vi "Confirm With User.vi"(8 "error in":errorcluster, 10 "message":string, 11 "key":string) -> (0 "error out":errorcluster, 1 "not supported?":bool, 2 "pending?":bool, 3 "confirmed?":bool)   [LabVIEW 2020, in "MCP Server.lvlib"]
doc: "Asks the user of the MCP client to confirm something (MCP elicitation without fields), for example before a tool deletes data or moves hardware. A wrapper around Ask User.vi with an empty requestedSchema.\n\nThe tool VI runs twice: on the first run pending? is TRUE - return at once and do NOTHING else, no side effects. On the second run confirmed? is TRUE when the user accepted; when it is FALSE (and pending? and not supported? are FALSE) the user declined or cancelled. not supported? is TRUE when the client cannot be asked (a legacy client, or no elicitation capability): fall back to a safe default or refuse.\n\nkey must be unique within the tool. See Ask User.vi for the details and the restrictions of form mode (never ask for passwords or keys)."
uses:
  MCP Server.lvlib
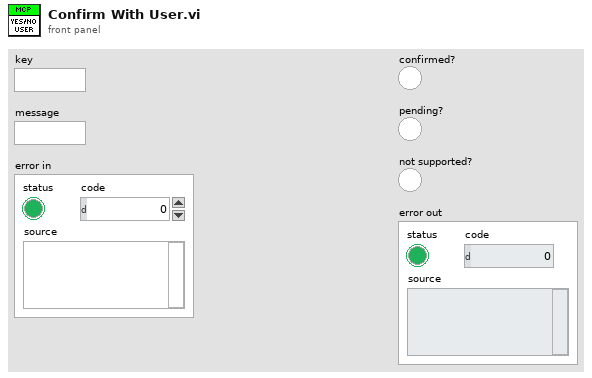
[diagram p1: front panel]
types:
  T1 = enum16{"accept", "decline", "cancel", "pending", "not supported"}
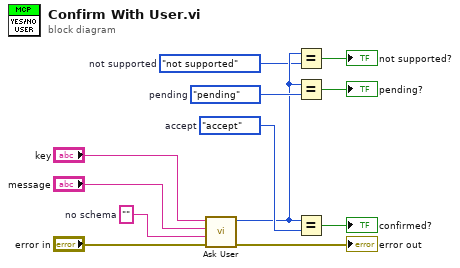
[diagram p0: block diagram]
diagram:
  w3 = T1."not supported"  # not supported
  w6 = T1."pending"  # pending
  w8 = T1."accept"  # accept
  w10 = ""  # no schema
  n1 = call "Ask User.vi"("error in"="error in", "requestedSchema"=w10, "message"="message", "key"="key") -> ("error out"=→"error out":errorcluster, "action"=w4:T1)  [unwired: 5 in, 1 out]
  n2 = Equal?(x=w4, y=w3) -> (x = y?=→"not supported?":bool)
  n3 = Equal?(x=w4, y=w6) -> (x = y?=→"pending?":bool)
  n4 = Equal?(x=w4, y=w8) -> (x = y?=→"confirmed?":bool)
